vi "Pre-Build VI - Run Unit Tests.vi"(8 "error in (no error)":errorcluster) -> (0 "error out":errorcluster, 1 "VIs without test coverage":string[](array[string]), 2 "error type":enum16{"fatal", "non-fatal", "warning"}(ring))   [LabVIEW 2009]
uses:
  <userlib>/_OpenG.lib/array/array.llb/Empty 1D Array (String)__ogtk.vi
  <userlib>/_OpenG.lib/array/array.llb/Filter 1D Array (String)__ogtk.vi
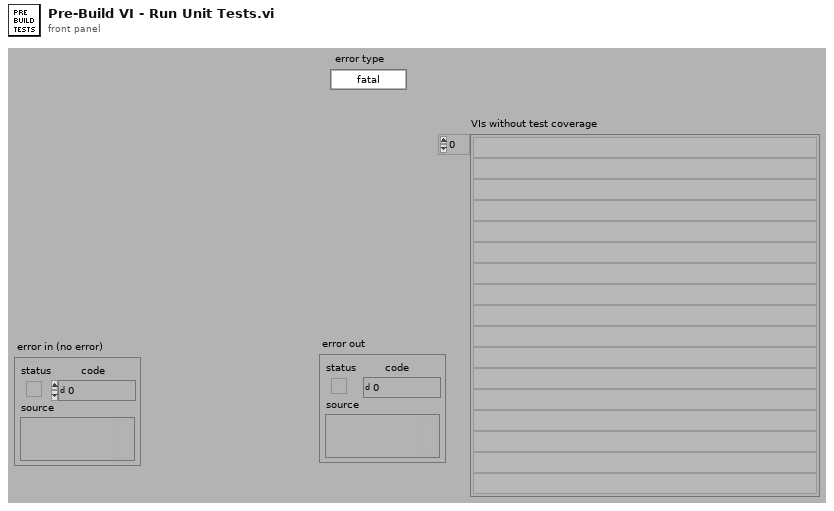
[diagram p1: front panel]
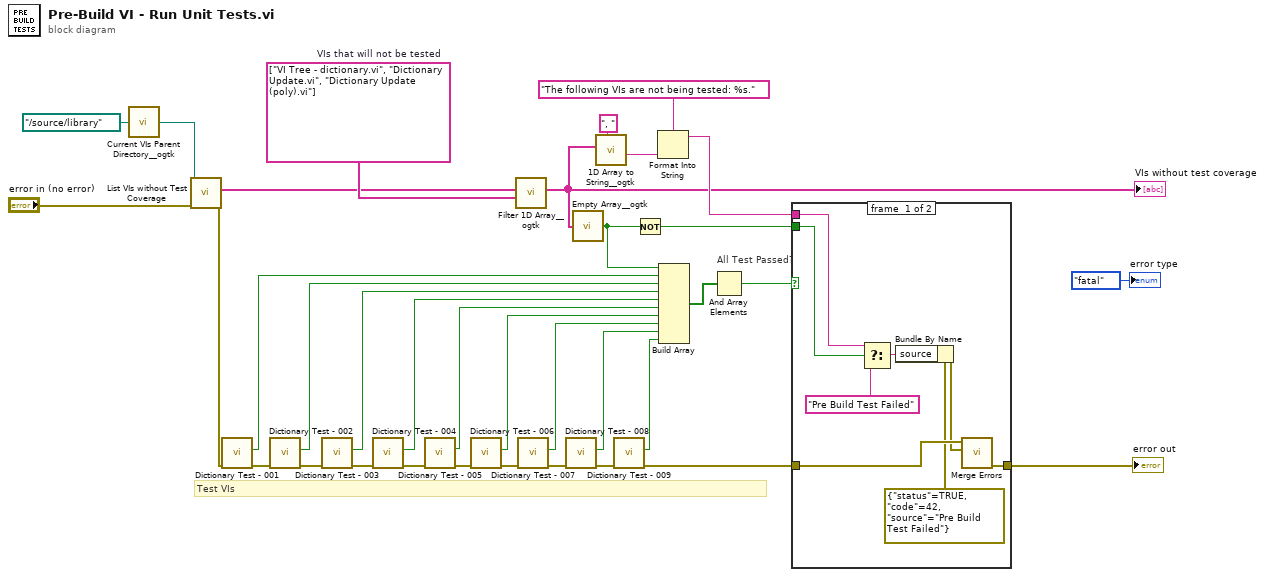
[diagram p0: block diagram]
diagram:
  w27 = string[] ["VI Tree - dictionary.vi", "Dictionary Update.vi", "Dictionary Update (poly).vi"]  # VIs that will not be tested
  # "All Test Passed?"
  # "Test VIs"
  n1 = call <userlib>:"Current VIs Parent Directory__ogtk.vi"("Relative path (.)"=path "../source/library") -> ("Parent Directory (+ Relative)"=w2:path)  [unwired: 4 in]
  n2 = call "List VIs without Test Coverage.vi"("error in (no error)"="error in (no error)", "Source Root"=w2) -> ("error out"=w28:errorcluster, "VIs without test coverage"=w26:string[])  [unwired: 8 in]
  n3 = call "Dictionary Test - 001.vi"("error in (no error)"=w28) -> ("error out"=w30:errorcluster, "pass"=w34:bool)  [unwired: 9 in]
  n4 = call "Dictionary Test - 002.vi"("error in (no error)"=w30) -> ("error out"=w19:errorcluster, "pass"=w29:bool)  [unwired: 9 in]
  n5 = call "Dictionary Test - 003.vi"("error in (no error)"=w19) -> ("error out"=w17:errorcluster, "pass"=w18:bool)  [unwired: 9 in]
  n6 = call "Dictionary Test - 004.vi"("error in (no error)"=w17) -> ("error out"=w14:errorcluster, "pass"=w16:bool)  [unwired: 9 in]
  n7 = call "Dictionary Test - 005.vi"("error in (no error)"=w14) -> ("error out"=w13:errorcluster, "pass"=w11:bool)  [unwired: 9 in]
  n8 = call "Dictionary Test - 006.vi"("error in (no error)"=w13) -> ("error out"=w12:errorcluster, "pass"=w10:bool)  [unwired: 9 in]
  n9 = call-poly <userlib>:"Filter 1D Array__ogtk.vi"("Items to Filter"=w27, "String Array"=w26) -> ("Filtered String Array"=w3:string[])  [unwired: 5 in]
  "VIs without test coverage" <- w3
  n10 = call "Dictionary Test - 007.vi"("error in (no error)"=w12) -> ("error out"=w8:errorcluster, "pass"=w9:bool)  [unwired: 9 in]
  n11 = call "Dictionary Test - 008.vi"("error in (no error)"=w8) -> ("error out"=w7:errorcluster, "pass"=w5:bool)  [unwired: 9 in]
  n12 = call-poly <userlib>:"Empty Array__ogtk.vi"("Array"=w3) -> ("Empty Array?"=w21:bool)  [unwired: 8 in]
  n13 = call <userlib>:"1D Array to String__ogtk.vi"("delimiter (Tab)"=", ", "Array of Strings"=w3) -> ("delimited string"=w24:string)  [unwired: 9 in]
  n14 = call "Dictionary Test - 009.vi"("error in (no error)"=w7) -> ("error out"=w6:errorcluster, "pass"=w4:bool)  [unwired: 9 in]
  n15 = Not(x=w21) -> (.not. x?=w20:bool)
  n16 = Format Into String(format string="The following VIs are not being tested: %s.", w24) -> (resulting string=w22:string)  [unwired: 2 in, 1 out]
  n17 = Build Array(w21, w34, w29, w18, w16, w11, w10, w9, w5, w4) -> (w33:bool[])
  n18 = And Array Elements(Boolean array=w33) -> (logical AND=w32:bool)
  n19 = case shown="False" w32 {
    tunnel: w6 -> [w43 w44]
    tunnel: [w42 w44] -> w31
    tunnel: w20 -> [w41 _]
    tunnel: w22 -> [w40 _]
    frame #0 {
      n20 = Select(t=w40, s=w41, f="Pre Build Test Failed" ("source")) -> (s? t:f=w38:string)
      n21 = Bundle By Name(cluster=errorcluster {"status"=TRUE, "code"=42, "source"="Pre Build Test Failed"} ("error out"), "source"=w38) -> (w37:errorcluster)
      n22 = call <vilib>:"Merge Errors.vi"("error in 2 (no error)"=w37, "error in 1 (no error)"=w43) -> ("error out"=w42:errorcluster)  [unwired: 5 in]
    }
    frame #1 {
    }
  }
  "error out" <- w31
  "error type" <- enum16{"fatal", "non-fatal", "warning"}."fatal" ("error type")
